vi "Unregister MessageQ.vi"(8 "error in (no error)":errorcluster, 11 "Module in":refnum<class "Module.lvclass">) -> (0 "error out":errorcluster, 3 "Module out":refnum<class "Module.lvclass">)   [LabVIEW 2020, in "Volatus.lvlib" / "Module.lvclass"]
uses:
  Module.lvclass
  Remote Messaging Identity/Remote Messaging Identity.lvclass
  C:/dev/lv20CE/relink/lv-volatus/Volatus/Identity/Identity.lvclass
  Message Unregistration.ctl
  MessageQ/MessageQ.lvclass
  Module.lvclass/Module.ctl
  MessageQ/MessageQ.lvclass/MessageQ.ctl
  VolatusAPI/VolatusAPI.lvclass
  Volatus.lvlib
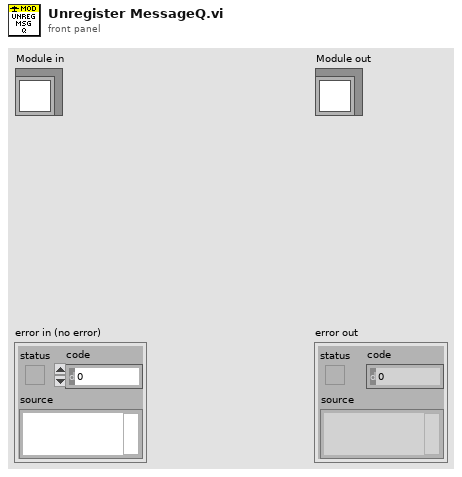
[diagram p1: front panel]
types:
  T1 = typedef "Volatus.lvlib/Message Unregistration.ctl" = cluster{"MessageQ":refnum<class "MessageQ.lvclass">}
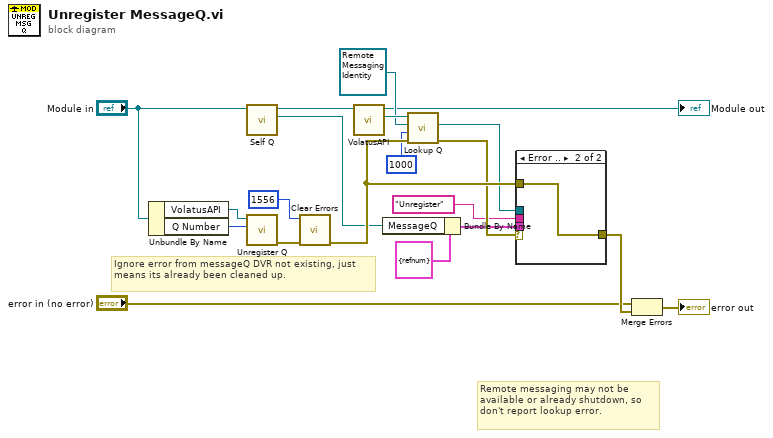
[diagram p0: block diagram]
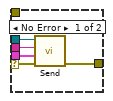
[diagram p2: hidden frame]
diagram:
  # "Ignore error from messageQ DVR not existing, just means its already been cleaned up."
  # "Remote messaging may not be available or already shutdown, so don't report lookup error."
  n1 = Unbundle By Name("Module in") -> ("VolatusAPI"=w17:refnum<class "VolatusAPI.lvclass">, "Q Number"=w16:i32)
  n2 = call "Self Q.vi"("Module in"="Module in") -> ("Self Q"=w5:refnum<class "MessageQ.lvclass">, "Module out"=w13:refnum<class "Module.lvclass">)  [unwired: 9 in]
  n3 = call "Unregister Q.vi"("Q Number"=w16, "VolatusAPI in"=w17) -> ("error out"=w19:errorcluster)  [unwired: 8 in, 1 out]
  n4 = call <vilib>:"Clear Errors.vi"("error in (no error)"=w19, "specific error code to clear (0: all)"=1556) -> ("error out"=w20:errorcluster)  [unwired: 4 in, 1 out]
  n5 = call "VolatusAPI.vi"("Module in"=w13) -> ("VolatusAPI"=w15:refnum<class "VolatusAPI.lvclass">, "Module out"=→"Module out":refnum<class "Module.lvclass">)  [unwired: 9 in]
  n6 = Bundle By Name(cluster=T1 {"MessageQ"=refnum} ("Message Unregistration"), "MessageQ"=w5) -> (w6:T1)
  n7 = call "Lookup Q.vi"("error in (no error)"=w20, "Timeout ms (0)"=1000, "Identity"=refnum<class "Remote Messaging Identity.lvclass"> refnum ("Volatus:Remote Messaging Identity.lvclass"), "VolatusAPI in"=w15) -> ("error out"=w11:errorcluster, "MessageQ"=w9:refnum<class "MessageQ.lvclass">)  [unwired: 5 in, 1 out]
  n8 = case shown="Error .." w11 {
    selector: w11 -> [w25 _]
    tunnel: [w24 w26] -> w10
    tunnel: w9 -> [w23 _]
    tunnel: "Unregister" ("ID") -> [w22 _]
    tunnel: w6 -> [w21 _]
    tunnel: w20 -> [_ w26]
    frame No Error {
      n9 = call "Send.vi"("error in (no error)"=w25, "Data"=w21, "ID"=w22, "MessageQ in"=w23) -> ("error out"=w24:errorcluster)  [unwired: 6 in, 1 out]
    }
    frame Error {
    }
  }
  n10 = Merge Errors("error in (no error)", w10) -> (→"error out":errorcluster)
